vi "Host_Writes.vi"(2 "Prev Fault":u16, 4 "Clear Bin":bool, 5 "Bin Full":bool, 6 "E-Stop":bool, 7 "Clamp Stuck":bool, 8 "Reset":bool, 9 "Stop":bool, 10 "Start":bool, 11 "Queue":refnum<queue>) -> (3 "Fault":u16)   [LabVIEW 2018]
doc: "Use this template to build a VI to use as a subVI."
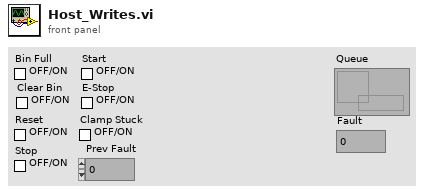
[diagram p1: front panel]
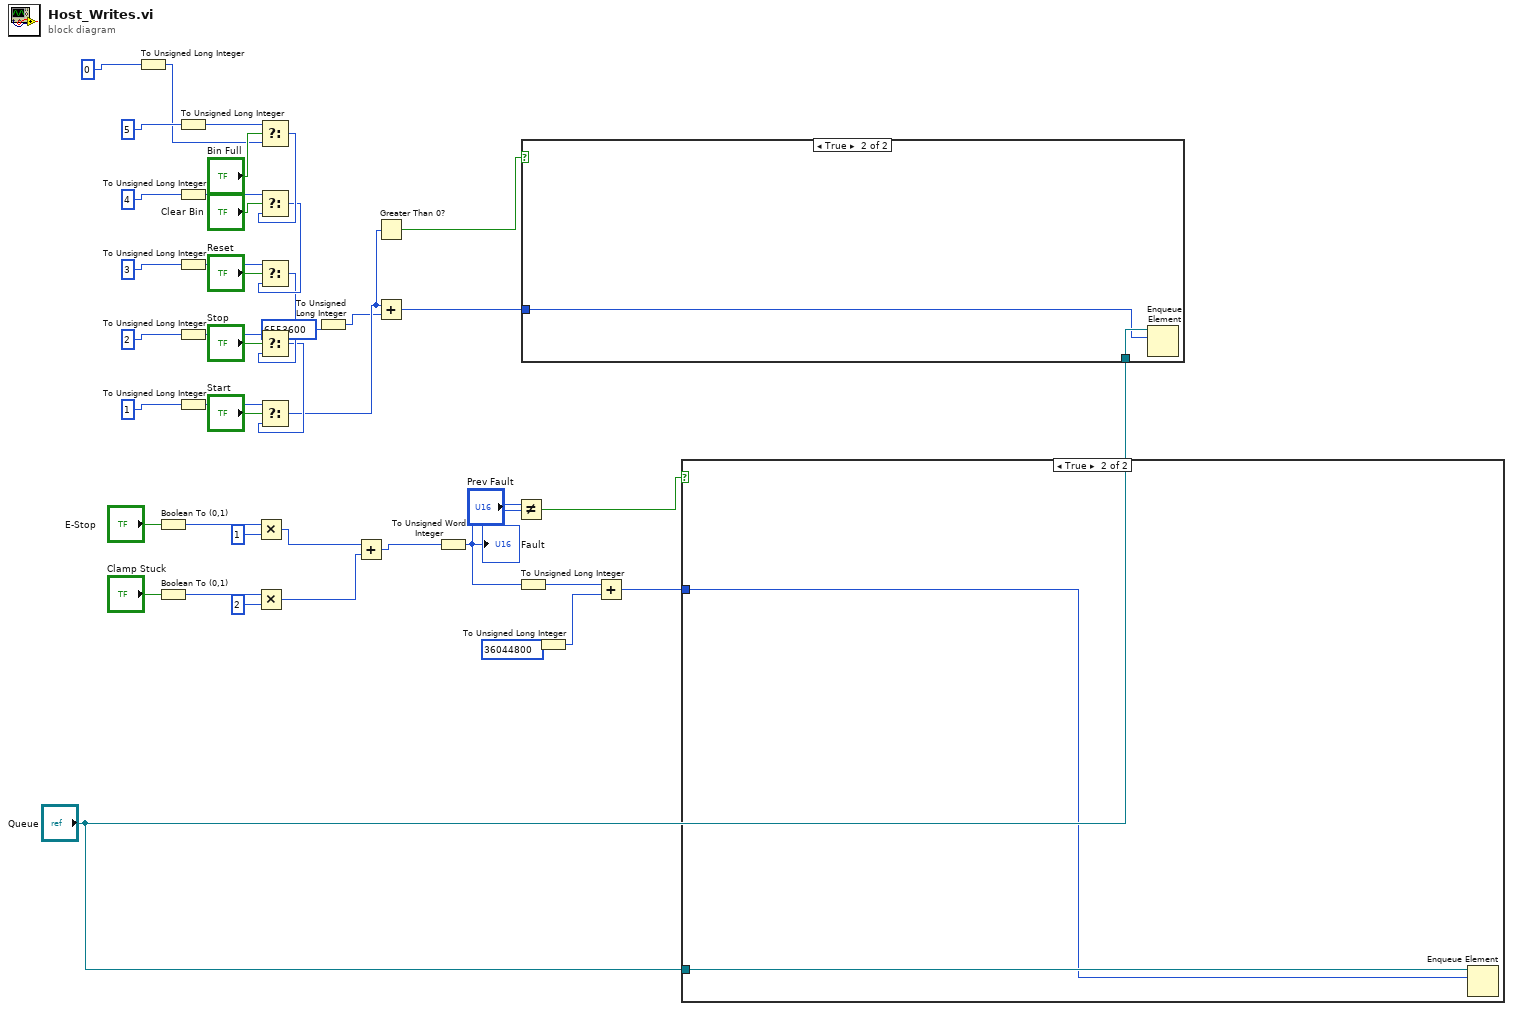
[diagram p0: block diagram]
diagram:
  n1 = To Unsigned Long Integer(number=0) -> (unsigned 32bit integer=w39:u32)
  n2 = Boolean To (0,1)(Boolean="E-Stop") -> (0, 1=w16:i16)
  n3 = Boolean To (0,1)(Boolean="Clamp Stuck") -> (0, 1=w13:i16)
  n4 = To Unsigned Long Integer(number=5) -> (unsigned 32bit integer=w40:u32)
  n5 = To Unsigned Long Integer(number=4) -> (unsigned 32bit integer=w36:u32)
  n6 = To Unsigned Long Integer(number=3) -> (unsigned 32bit integer=w32:u32)
  n7 = To Unsigned Long Integer(number=2) -> (unsigned 32bit integer=w28:u32)
  n8 = To Unsigned Long Integer(number=1) -> (unsigned 32bit integer=w24:u32)
  n9 = Multiply(x=w16, y=i16 1) -> (x*y=w11:i16)
  n10 = Multiply(x=w13, y=i16 2) -> (x*y=w10:i16)
  n11 = Select(t=w40, s="Bin Full", f=w39) -> (s? t:f=w35:u32)
  n12 = Select(t=w36, s="Clear Bin", f=w35) -> (s? t:f=w31:u32)
  n13 = Select(t=w32, s="Reset", f=w31) -> (s? t:f=w27:u32)
  n14 = Select(t=w28, s="Stop", f=w27) -> (s? t:f=w23:u32)
  n15 = Select(t=w24, s="Start", f=w23) -> (s? t:f=w22:u32)
  n16 = To Unsigned Long Integer(number=6553600) -> (unsigned 32bit integer=w20:u32)
  n17 = Add(x=w11, y=w10) -> (x+y=w9:i16)
  n18 = Greater Than 0?(x=w22) -> (x > 0?=w19:bool)
  n19 = Add(x=w22, y=w20) -> (x+y=w18:u32)
  n20 = To Unsigned Word Integer(number=w9) -> (unsigned 16bit integer=w8:u16)
  "Fault" <- w8
  n21 = Not Equal?(x=w8, y="Prev Fault") -> (x != y?=w3:bool)
  n22 = To Unsigned Long Integer(number=w8) -> (unsigned 32bit integer=w6:u32)
  n23 = case shown="True" w19 {
    tunnel: "Queue" -> [_ w45]
    tunnel: w18 -> [_ w44]
    frame False {
    }
    frame True {
      n24 = Enqueue Element(queue=w45, element=w44) -> ()  [unwired: 2 in, 3 out]
    }
  }
  n25 = To Unsigned Long Integer(number=36044800) -> (unsigned 32bit integer=w4:u32)
  n26 = Add(x=w6, y=w4) -> (x+y=w1:u32)
  n27 = case shown="True" w3 {
    tunnel: "Queue" -> [_ w47]
    tunnel: w1 -> [_ w46]
    frame False {
    }
    frame True {
      n28 = Enqueue Element(queue=w47, element=w46) -> ()  [unwired: 2 in, 3 out]
    }
  }
